vi "create default cache.vi"() -> (3 "cache":T1)   [LabVIEW 2013, in "PL_class cache.lvlib"]
uses:
  PL_class cache.lvlib
  cache definition.ctl
  cache search configuration.ctl
  cached class information.ctl
  target class metadata.ctl
  class metadata.ctl
  <vilib>/NI/Tag Bus Module Framework/root configuration/Target Types.ctl
  <vilib>/Utility/libraryn.llb/Check if File or Folder Exists.vi
  <vilib>/NI/Tag Bus Module Framework/root configuration/TBM configuration.lvclass
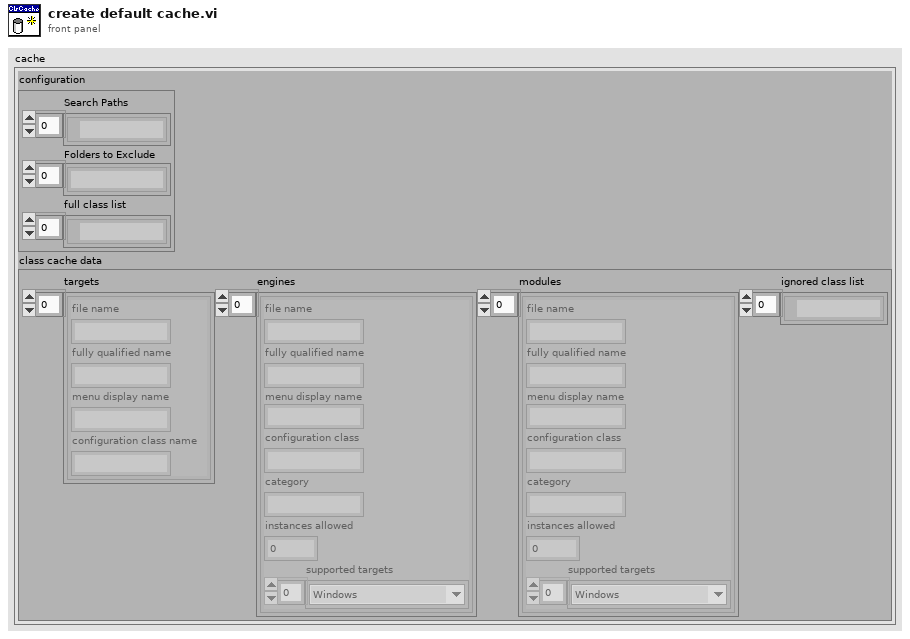
[diagram p1: front panel]
types:
  T1 = typedef "PL_class cache.lvlib/cache definition.ctl" = cluster{"configuration":T2, "class cache data":T3}
  T2 = typedef "PL_class cache.lvlib/cache search configuration.ctl" = cluster{"Search Paths":path[], "Folders to Exclude":string[], "full class list":path[]}
  T3 = typedef "PL_class cache.lvlib/cached class information.ctl" = cluster{"targets":T4[], "engines":T5[], "modules":T5[], "ignored class list":path[]}
  T4 = typedef "PL_class cache.lvlib/target class metadata.ctl" = cluster{"file name":string, "fully qualified name":string, "menu display name":string, "configuration class name":string}
  T5 = typedef "PL_class cache.lvlib/class metadata.ctl" = cluster{"file name":string, "fully qualified name":string, "menu display name":string, "configuration class":string, "category":string, "instances allowed":i32, "supported targets":T6[]}
  T6 = typedef "TBM configuration.lvclass/Target Types.ctl" = enum16{"Windows", "Mac", "Linux", "Linux RT ARM", "VxWorks", "Pharlap", "Other", "Linux RT x64"}
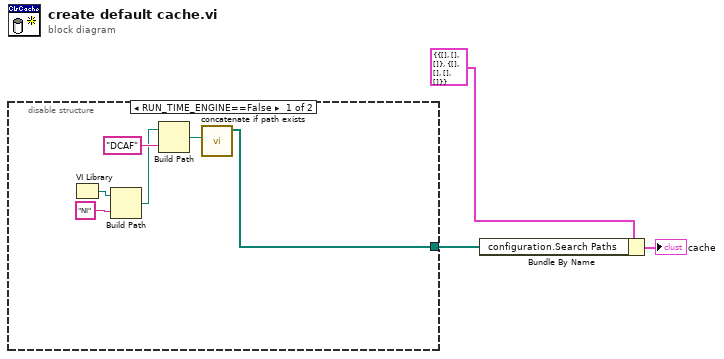
[diagram p0: block diagram]
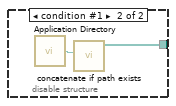
[diagram p2: hidden frame]
diagram:
  n1 = disable-structure shown="RUN_TIME_ENGINE==False" {
    disable-tunnel: [w4 w10] -> w3
    frame condition #0 (active) {
      n2 = VI Library() -> (path=w9:path)
      n3 = Build Path(base path=w9, name or relative path="NI") -> (appended path=w5:path)
      n4 = Build Path(base path=w5, name or relative path="DCAF") -> (appended path=w6:path)
      n5 = call "concatenate if path exists.vi"("new path"=w6) -> ("paths out"=w4:path[])  [unwired: 10 in]
    }
    frame condition #1 {
      n6 = call <vilib>:"Application Directory.vi"() -> ("Application Directory"=w11:path)
      n7 = call "concatenate if path exists.vi"("new path"=w11) -> ("paths out"=w10:path[])  [unwired: 10 in]
    }
  }
  n8 = Bundle By Name(cluster=T1 {"configuration"={"Search Paths"=[], "Folders to Exclude"=[], "full class list"=[]}, "class cache data"={"targets"=[], "engines"=[], "modules"=[], "ignored class list"=[]}} ("cache"), "configuration.Search Paths"=w3) -> (→"cache":T1)
